vi "ImplicitParameterNode_Create.vi"(0 "reference":refnum<class "ImplicitParameterNode.lvclass">, 5 "error in (no error)":errorcluster) -> (14 "reference out":refnum<class "ImplicitParameterNode.lvclass">, 19 "error out":errorcluster)   [LabVIEW 2020, in "ImplicitParameterNode.lvclass"]
doc: "Creates and initializes a new ImplicitParameterNode object.\n\nThis object should be destroyed using a ImplicitParameterNode destructor VI or a virtual base class destructor VI.\n\n[GOOP 2.3]"
uses:
  <resource>/Framework/Providers/Open_GDS/UML/ImplicitParameterNode_class/ImplicitParameterNode.lvclass
  C:/Program Files (x86)/National Instruments/LabVIEW 2020/resource/Framework/Providers/Open_GDS/UML/RectangularNode_class/RectangularNode.lvclass
  <resource>/Framework/Providers/Open_GDS/UML/General/Rectangle/Rectangle Rectangle2D.ctl
  <resource>/Framework/Providers/Open_GDS/UML/RectangularNode_class/RectangularNode.lvclass
  <resource>/Framework/Providers/Open_GDS/UML/MultiLineString_class/MultiLineString.lvclass
panel:
  # "The input reference should only\nbe wired when this method is called\nby a sub class constructor."
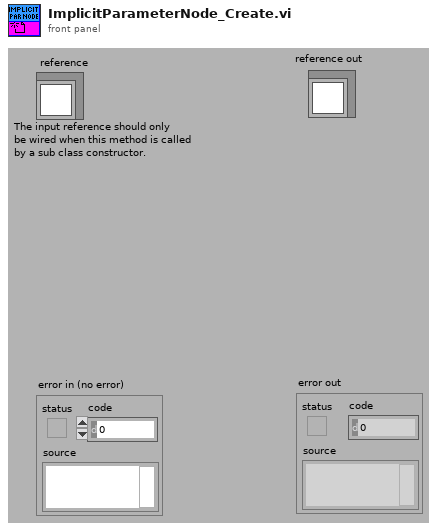
[diagram p1: front panel]
types:
  T1 = typedef "Rectangle Rectangle2D.ctl" = cluster{"x":dbl, "y":dbl, "width":dbl, "height":dbl}
  T2 = typedef "ImplicitParameterNode.lvclass/ObjectAttributes.ctl" = cluster{"topHeight":dbl, "name":refnum<class "MultiLineString.lvclass">, "DEFAULT_TOP_HEIGHT":i32, "DEFAULT_WIDTH":i32, "DEFAULT_HEIGHT":i32}
  T3 = typedef "RectangularNode.lvclass/ObjectAttributes.ctl" = cluster{"bounds":T1}
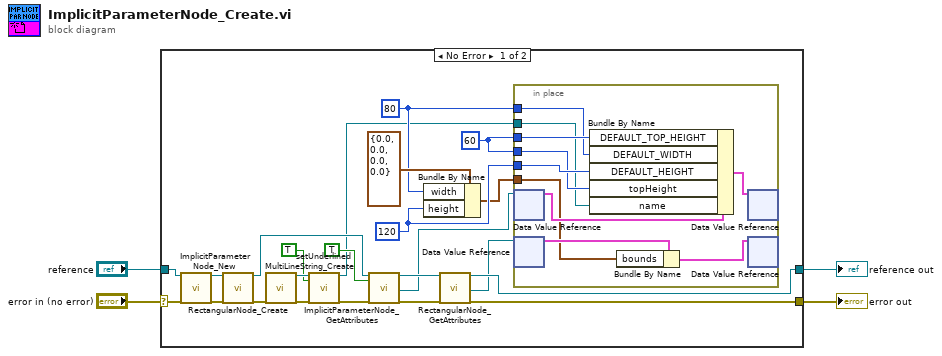
[diagram p0: block diagram]
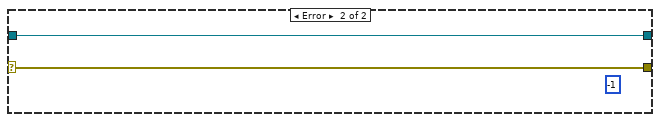
[diagram p2: hidden frame]
diagram:
  n1 = case shown="No Error" "error in (no error)" {
    selector: "error in (no error)" -> [w27 w39]
    tunnel: [w22 w38] -> w4
    tunnel: [w21 w39] -> w3
    tunnel: "reference" -> [w26 w38]
    frame No Error {
      w8 = 120 ("DEFAULT_HEIGHT")
      w9 = 80 ("DEFAULT_WIDTH")
      w7 = 60 ("DEFAULT_TOP_HEIGHT")
      n2 = call <resource>:"ImplicitParameterNode_New.vi"("reference in"=w26, "error in (no error)"=w27) -> ("reference out"=w24:refnum<class "ImplicitParameterNode.lvclass">, "error out"=w25:errorcluster)  [unwired: 2 in, 14 out]
      n3 = call <resource>:"RectangularNode_Create.vi"("reference"=w24, "error in (no error)"=w25) -> ("reference out"=w23:refnum<class "ImplicitParameterNode.lvclass">, "error out"=w20:errorcluster)  [unwired: 1 in, 15 out]
      n4 = call <resource>:"MultiLineString_Create.vi"("error in (no error)"=w20) -> ("reference out"=w19:refnum<class "MultiLineString.lvclass">, "error out"=w18:errorcluster)  [unwired: 2 in, 15 out]
      n5 = call <resource>:"setUnderlined.vi"("reference"=w19, "underlined"=TRUE, "error in (no error)"=w18) -> ("reference out"=w6:refnum<class "MultiLineString.lvclass">, "error out"=w16:errorcluster)  [unwired: 15 out]
      n6 = call <resource>:"ImplicitParameterNode_GetAttributes.vi"("reference in"=w23, "OnlyGetDvrReference(False)"=TRUE, "error in (no error)"=w16) -> ("reference out"=w13:refnum<class "ImplicitParameterNode.lvclass">, "DataRef"=w11:refnum<data-value>, "error out"=w12:errorcluster)  [unwired: 13 in, 1 out]
      n7 = Bundle By Name(cluster=T1 {"x"=0.0, "y"=0.0, "width"=0.0, "height"=0.0} ("Base class.bounds"), "width"=w9, "height"=w8) -> (w5:T1)
      n8 = call <resource>:"RectangularNode_GetAttributes.vi"("reference in"=w13, "error in (no error)"=w12) -> ("reference out"=w22:refnum<class "ImplicitParameterNode.lvclass">, "DataRef"=w10:refnum<data-value>, "error out"=w21:errorcluster)  [unwired: 14 in, 1 out]
      n9 = in-place {
        in-place-border: w7 -> [w36]
        in-place-border: w9 -> [w35]
        in-place-border: w8 -> [w34]
        in-place-border: w7 -> [w33]
        in-place-border: w6 -> [w32]
        in-place-border: w5 -> [w29]
        n10 = in-place-dvr #1(w11) -> (w37:T2)  [unwired: 1 out]
        n11 = in-place-dvr #2(w10) -> (w30:T3)  [unwired: 1 out]
        n12 = Bundle By Name(cluster=w37, "DEFAULT_TOP_HEIGHT"=w36, "DEFAULT_WIDTH"=w35, "DEFAULT_HEIGHT"=w34, "topHeight"=w33, "name"=w32) -> (w31:T2)
        n13 = Bundle By Name(cluster=w30, "bounds"=w29) -> (w28:T3)
        n14 = in-place-dvr #1(w31) -> ()  [unwired: 2 out]
        n15 = in-place-dvr #2(w28) -> ()  [unwired: 2 out]
      }
    }
    frame Error {
      (unwired) -1 ("Nr of open handles")
    }
  }
  "error out" <- w3
  "reference out" <- w4
